vi "RDC-Lin-Compensate_Calc_Permittivity.vi"(5 "C0":dbl, 7 "Tau":dbl format="%#_6e", 10 "input cluster":T1) -> (2 "Output cluster":T1)   [LabVIEW 2020, in "RDC-Reflection_Data_Computation.lvlib"]
doc: "Corrects the reflection of a Common Format cluster with Tau, computes the impedance and then the permittivity with C0. Returns the cluster with the computed values."
uses:
  RDC-Reflection_Data_Computation.lvlib
  Reflector/RFH-common_data_format.ctl
  Reflector/RFH-Reflection_File_Handler.lvlib
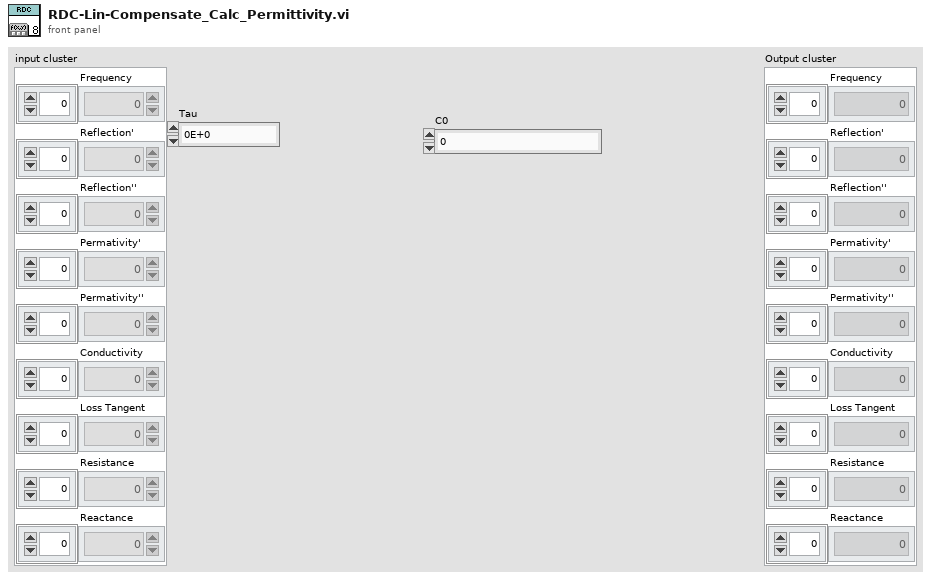
[diagram p1: front panel]
types:
  T1 = typedef "RFH-Reflection_File_Handler.lvlib/RFH-common_data_format.ctl" = cluster{"Frequency":dbl[], "Reflection'":dbl[], "Reflection''":dbl[], "Permativity'":dbl[], "Permativity''":dbl[], "Conductivity":dbl[], "Loss Tangent":dbl[], "Resistance":dbl[], "Reactance":dbl[]}
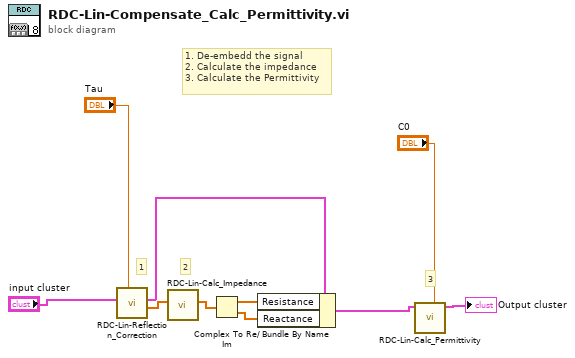
[diagram p0: block diagram]
diagram:
  # "1. De-embedd the signal\n2. Calculate the impedance\n3. Calculate the Permittivity"
  # "3"
  # "2"
  # "1"
  n1 = call "RDC-Lin-Reflection_Correction.vi"("Tau"="Tau", "Measured"="input cluster") -> ("Reflection Tip"=w9:cdb[], "Tip"=w7:T1)  [unwired: 8 in]
  n2 = call "RDC-Lin-Calc_Impedance.vi"("Reflection Tip"=w9) -> ("Impedance"=w6:cdb[])  [unwired: 9 in, 1 out]
  n3 = Complex To Re/Im(x + iy=w6) -> (x=w5:dbl[], y=w4:dbl[])
  n4 = Bundle By Name(cluster=w7, "Resistance"=w5, "Reactance"=w4) -> (w2:T1)
  n5 = call "RDC-Lin-Calc_Permittivity.vi"("C0"="C0", "input cluster"=w2) -> ("Output cluster"=→"Output cluster":T1)  [unwired: 9 in]
